vi "Start Logic-Mode dependent case 2.vi"(6 "Case name string":string, 8 "error in (no error)":errorcluster, 9 "cancelled":bool, 10 "UI queue":refnum<queue>, 11 "Acq. queue in":refnum<queue>) -> (0 "error out":errorcluster, 3 "Acq. queue out":refnum<queue>)   [LabVIEW 2017]
uses:
  Queue/Message Queue/Typedefs/Message Cluster.ctl
  Typedefs/Read Write Enum.ctl
  Typedefs/Top level VI states.ctl
  Global Variables/gl_UI Ctrl Refs.vi
  Global Variables/General Globals.vi
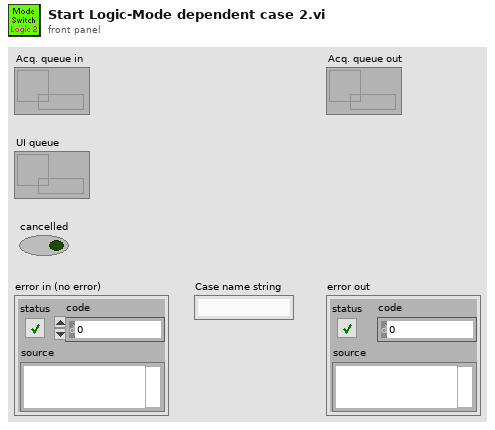
[diagram p1: front panel]
types:
  T1 = typedef "Read Write Enum.ctl" = enum16{"Read", "Write"}
  T2 = typedef "Top level VI states.ctl" = enum16{"None", "Initialise UI", "<STACK PROTOCOL STATES>", "AOL Zstack-START", "AOL Zstack-STOP", "Motor Zstack-START", "Motor Zstack-STOP", "Parameter Sweep-START", "Parameter Sweep-STOP", "<ACQUISITION PROTOCOL STATES> ", "Functional Acquisition-START", "Functional Acquisition-STOP", "Single Plane Acquisition-START", "Single Plane Acquisition-STOP", "Volume Acquisition-START", "Volume Acquisition-STOP", "<LIVE IMAGING PROTOCOL STATES>", "Live Imaging-START", "Live Imaging-STOP", "Live Plane Imaging-START", "Live Plane Imaging-STOP", "Live Volume Imaging-START", "Live Volume Imaging-STOP", "<MOVEMENT CORRECTION PROTOCOL STATES>", "EXIT"}
  T3 = typedef "UI ctrl refs cluster.ctl" = cluster{"Top level VI path":path, "Top level VI ref":refnum<vi>, "User menu ref":refnum<k9>, "Sub Panel control":refnum<vi>, "Imaging Param Tab":refnum<vi>, "Occurrence-Start drivers":refnum<k4>, "Occurrence-Speed logging initialised":refnum<k4>, "Occurrence-XYZ stage initialised":refnum<k4>, "Exit button":refnum<vi>, "Status ind":refnum<vi>, "Set as origin":refnum<vi>, "Speed Logging":refnum<vi>, "Time Lapse":refnum<vi>, "Live Imaging":refnum<vi>, "AOL Z Stack":refnum<vi>, "Motor Z Stack":refnum<vi>, "Funct Acq button":refnum<vi>, "Hard Shutter":refnum<vi>, "Virtual Shutter":refnum<vi>, "Laser Power":refnum<vi>, "AOL Mode":refnum<vi>, "Frame Size":refnum<vi>, "Field of View":refnum<vi>, "Dwell Time":refnum<vi>, "Zoom":refnum<vi>, "AOL Z":refnum<vi>, "Objective":refnum<vi>, "Axis":refnum<vi>, "Paths & Names":refnum<vi>, "Experiment folder path (ind.)":refnum<vi>, "Last State (Ind.)":refnum<vi>, "Averages":refnum<vi>, "Angle (degrees)":refnum<vi>, "X centre":refnum<vi>, "Y centre":refnum<vi>, "Plane Mode":refnum<vi>, "# Planes":refnum<vi>, "Z Start":refnum<vi>, "Z Stop":refnum<vi>, "Z Step":refnum<vi>, "PMT 1":refnum<vi>, "PMT 2":refnum<vi>, "Stage XYZ Position":refnum<vi>, "Pockels@Z Start":refnum<vi>, "Pockels@Z Stop":refnum<vi>, "Obtain Z Start":refnum<vi>, "Obtain Z Stop":refnum<vi>, "Live stim.trig.period":refnum<vi>, "Live stim.trig.enable":refnum<vi>, "Movement Correction":refnum<vi>, "Load Reference Image":refnum<vi>, "XY Stage Move":refnum<vi>, "MovCor Cluster":refnum<vi>, "RefDAQParam":refnum<vi>, "Funct. Acq. Pockels Modulation":refnum<vi>, "Ref Laser Power":refnum<vi>, "Enable Video Recording":refnum<vi>, "Video Record-Live Imaging":refnum<vi>, "Video Record-Funct acq":refnum<vi>, "Reference Source":refnum<vi>, "AOL Z-stack Chirps Ready (ind)":refnum<vi>, "Target time between mov.cor. ref triggers (ms)":refnum<vi>, "Funct. Acq. Ref frame save":refnum<vi>, "Tracking button":refnum<vi>, "Show ref plots window":refnum<vi>, "Center freq ind (nm)":refnum<vi>, "Pickup mode (ind)":refnum<vi>, "Logging queue (ind)":refnum<vi>, "Back aperture power (ind.)":refnum<vi>, "Power after objective (ind.)":refnum<vi>, "Switch user":refnum<vi>, "Ls1 Conn. Status":refnum<vi>, "Ls1Tuning Status":refnum<vi>, "Ls1 Faults":refnum<vi>, "Ls1 Connection":refnum<vi>, "Ls1 Mode":refnum<vi>, "Ls1 POWER [mW]":refnum<vi>, "Ls1Shutter":refnum<vi>, "Ls1 Wavelength":refnum<vi>, "Ls1 Note":refnum<vi>, "Ls1 Confirm Wav":refnum<vi>, "Ls1 PreChrp Prism1":refnum<vi>, "Ls1 PreChrp Prism2":refnum<vi>, "Ls1 wav top Ind":refnum<vi>, "Ls1 power top Ind":refnum<vi>, "Ls1 Pump peak Hold":refnum<vi>, "Ls1 Status Ind":refnum<vi>, "Ls1 wav cancel":refnum<vi>, "Experiment Type":refnum<vi>, "Biology Information":refnum<vi>, "Camera recording status":refnum<vi>, "# Sw. Planes":refnum<vi>, "Sweep Chirps ready":refnum<vi>, "Low-High Resolution Settings":refnum<vi>, "Parameter Sweep":refnum<vi>, "Sweep Chirps ready":refnum<vi>, "Start Sweep":refnum<vi>}
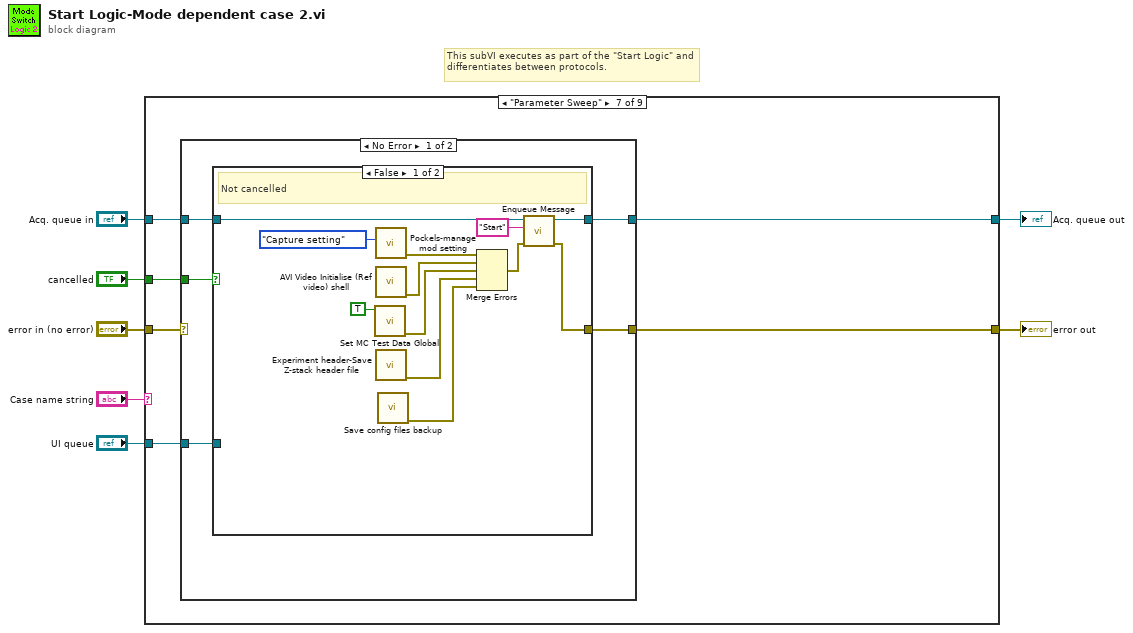
[diagram p0: block diagram]
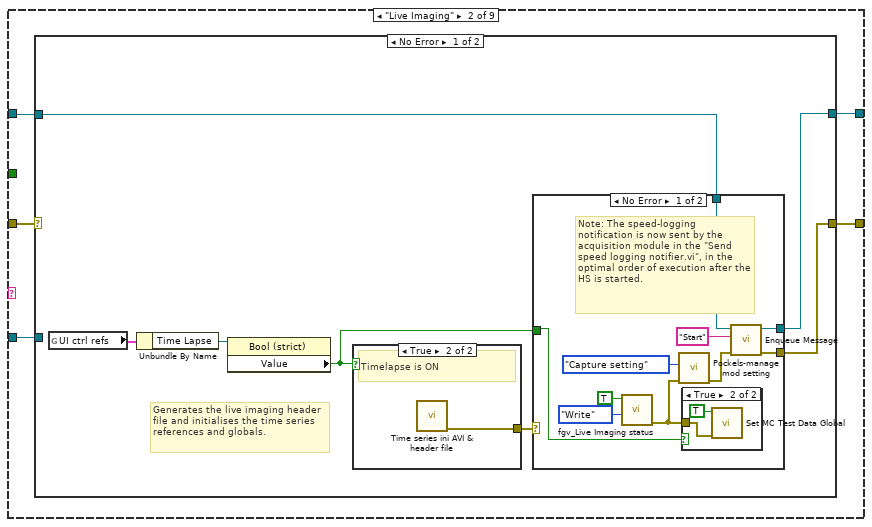
[diagram p3: hidden frame]
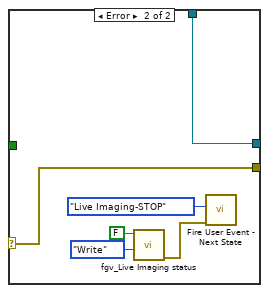
[diagram p5: hidden frame]
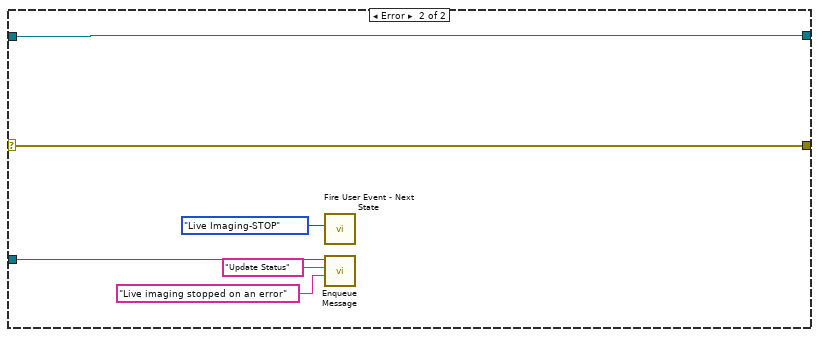
[diagram p7: hidden frame]
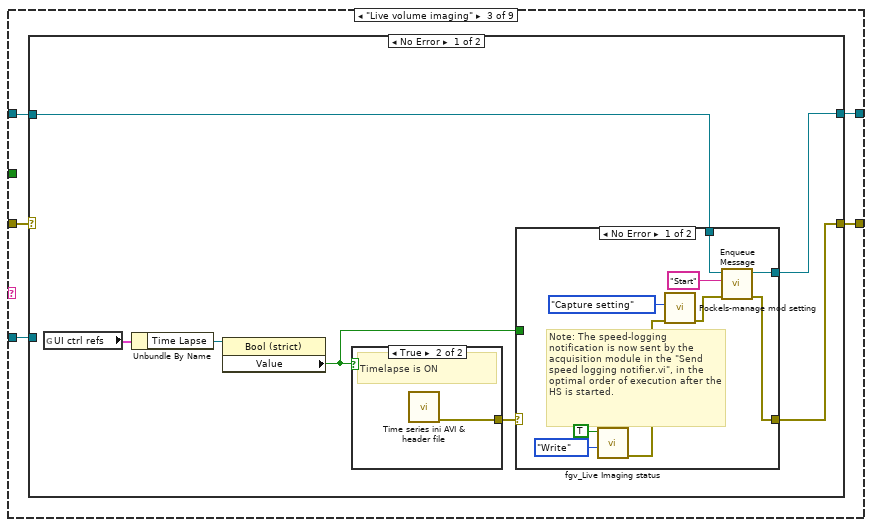
[diagram p8: hidden frame]
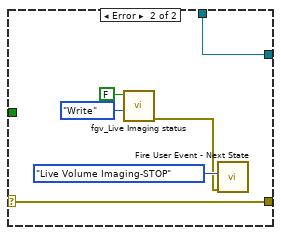
[diagram p9: hidden frame]
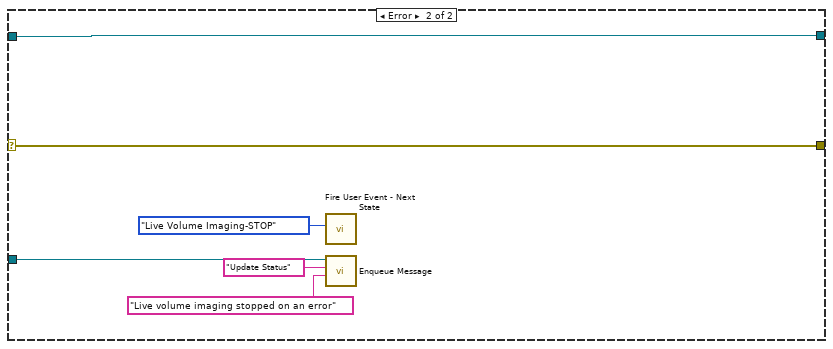
[diagram p11: hidden frame]
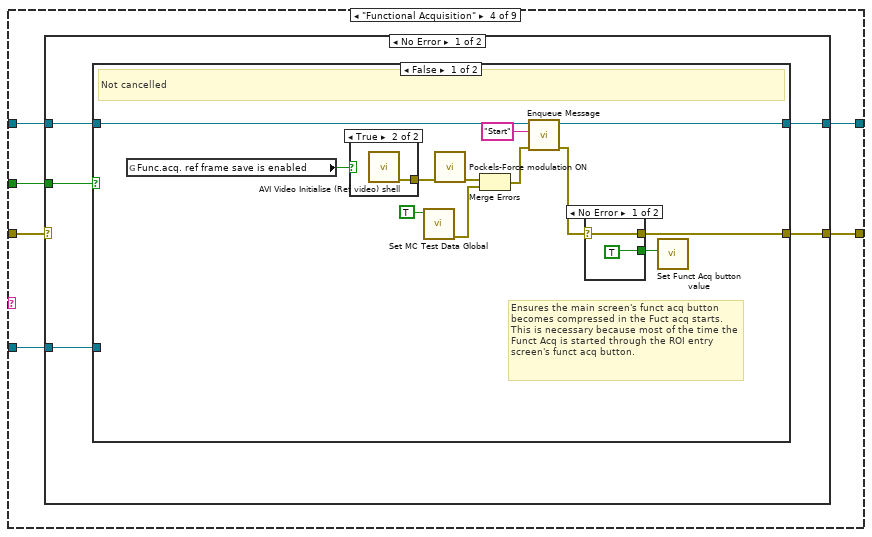
[diagram p12: hidden frame]
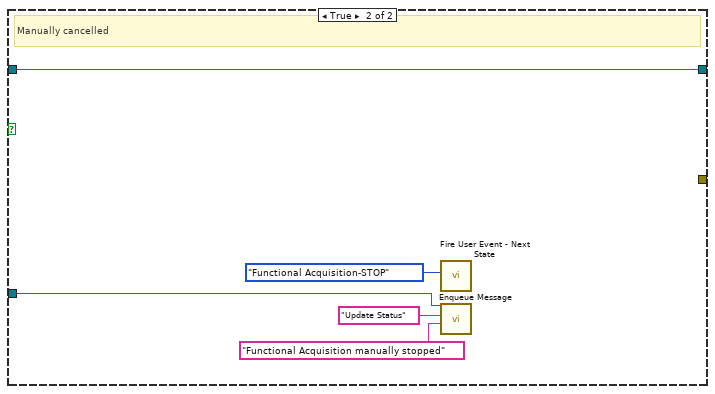
[diagram p15: hidden frame]
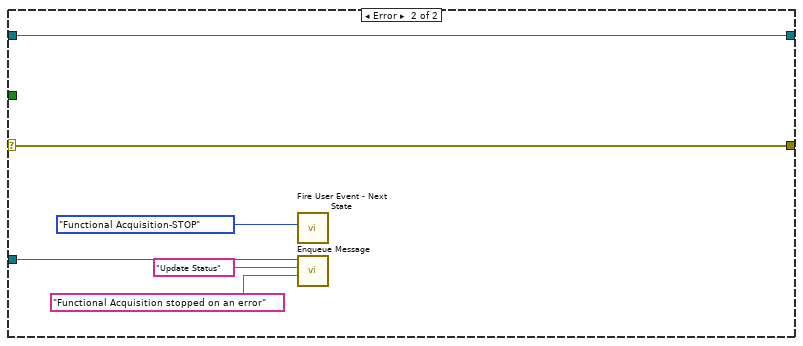
[diagram p16: hidden frame]
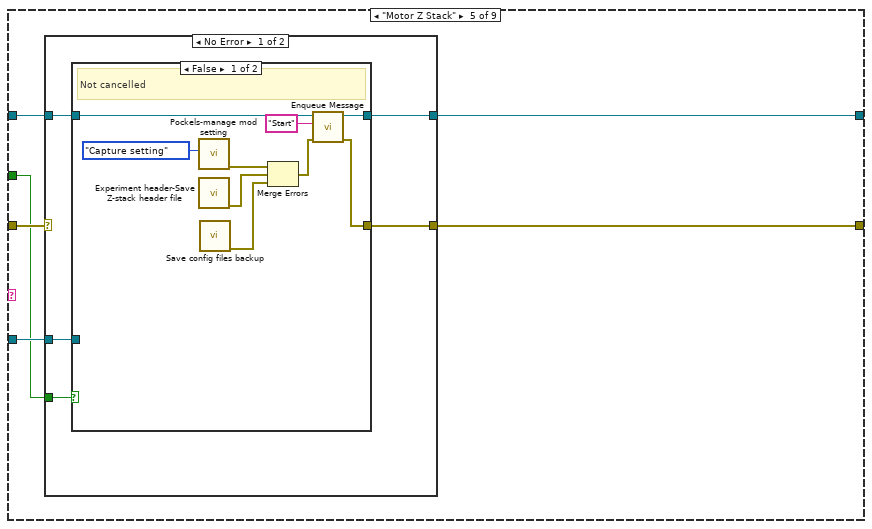
[diagram p17: hidden frame]
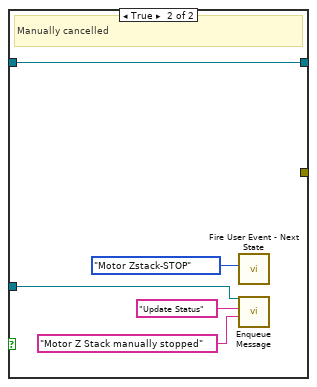
[diagram p18: hidden frame]
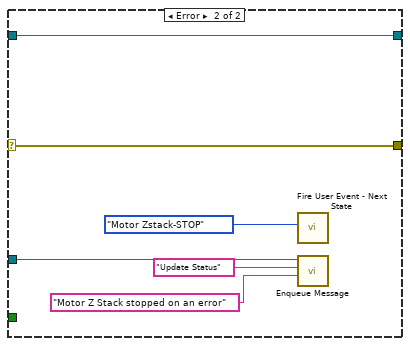
[diagram p19: hidden frame]
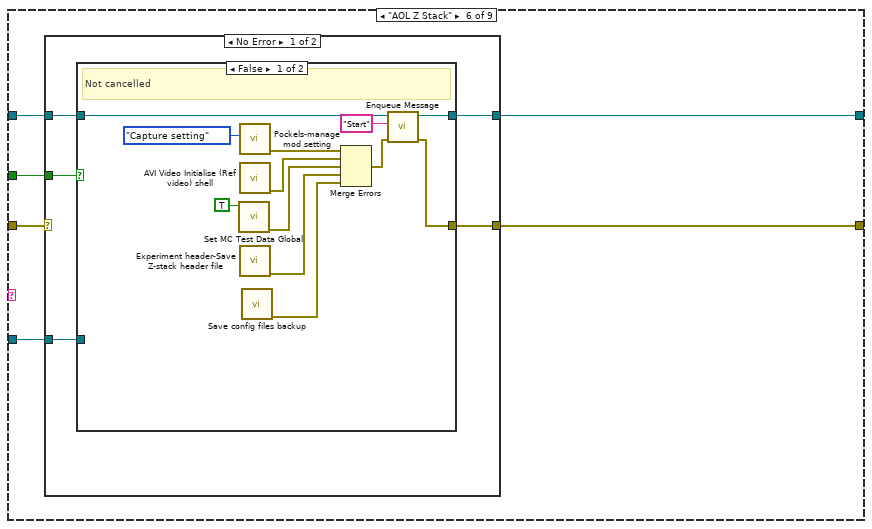
[diagram p20: hidden frame]
diagram:
  # "This subVI executes as part of the \"Start Logic\" and differentiates between protocols."
  n1 = case shown="\"Parameter Sweep\"" "Case name string" {
    tunnel: [w9 w14 w51 w83 w121 w152 w186 w220 w250] -> w1
    tunnel: "error in (no error)" -> [w9 w11 w48 w84 w122 w153 w187 w221 w251]
    tunnel: [w8 w12 w49 w86 w124 w155 w189 w223 w253] -> w3
    tunnel: "Acq. queue in" -> [w8 w13 w50 w85 w123 w154 w188 w222 w252]
    tunnel: "UI queue" -> [_ w10 w47 w82 w120 w151 w185 w219 w249]
    tunnel: "cancelled" -> [_ _ _ w81 w119 w150 w184 w218 w248]
    frame Default {
    }
    frame "Live Imaging" {
      n2 = case shown="No Error" w11 {
        selector: w11 -> [_ w46]
        tunnel: [w16 w46] -> w14
        tunnel: w13 -> [w18 w45]
        tunnel: [w17 w45] -> w12
        tunnel: w10 -> [_ w41]
        frame No Error {
          # "Generates the live imaging header file and initialises the time series references and globals."
          n3 = global read "gl_UI Ctrl Refs.vi" "UI ctrl refs"() -> (w15:T3)
          n4 = Unbundle By Name(w15) -> ("Time Lapse"=w21:refnum<vi>)
          n5 = property class="Bool (strict)"(reference=w21) -> ("Value"=w19:bool)  [unwired: 1 in, 2 out]
          n6 = case shown="True" w19 {
            tunnel: [_ w40] -> w20
            frame False {
              # "Timelapse is OFF"
            }
            frame True {
              # "Timelapse is ON"
              n7 = call "Time series ini AVI & header file.vi"() -> ("error out"=w40:errorcluster)  [unwired: 11 in]
            }
          }
          n8 = case shown="No Error" w20 {
            selector: w20 -> [_ w37]
            tunnel: w19 -> [w22 _]
            tunnel: w18 -> [w28 w38]
            tunnel: [w30 w38] -> w17
            tunnel: [w29 w37] -> w16
            frame No Error {
              # "Note: The speed-logging notification is now sent by the acquisition module in the \"Send speed logging notifier.vi\", in the optimal order of execution after the HS is started."
              n9 = call "fgv_Live Imaging status.vi"("Function"=Read_Write_Enum."Write", "Live Imaging?"=TRUE ("Timelapse?")) -> ("error out"=w23:errorcluster)  [unwired: 8 in, 1 out]
              n10 = call "Pockels-manage mod setting.vi"("error in (no error)"=w23, "Function"=enum16{"Capture setting", "Re-apply setting"}."Capture setting") -> ("error out"=w27:errorcluster)  [unwired: 9 in]
              n11 = case shown="True" w22 {
                tunnel: w23 -> [_ w32]
                frame False {
                }
                frame True {
                  n12 = call "Set MC Test Data Global.vi"("error in (no error)"=w32, "Save MC TestData"=TRUE) -> ()  [unwired: 8 in, 2 out]
                }
              }
              n13 = call "Enqueue Message.vi"("error in (no error)"=w27, "Message"="Start", "Queue"=w28) -> ("error out"=w29:errorcluster, "Queue out"=w30:refnum<queue>)  [unwired: 7 in]
            }
            frame Error {
              n14 = call "fgv_Live Imaging status.vi"("Function"=Read_Write_Enum."Write", "Live Imaging?"=FALSE ("Timelapse?")) -> ("error out"=w34:errorcluster)  [unwired: 8 in, 1 out]
              n15 = call "Fire User Event - Next State.vi"("Error In"=w34, "\"UI Handler loop\" case to execute"=Top_level_VI_states."Live Imaging-STOP" ("event data / imaging mode")) -> ()  [unwired: 9 in, 1 out]
            }
          }
        }
        frame Error {
          n16 = call "Fire User Event - Next State.vi"("\"UI Handler loop\" case to execute"=Top_level_VI_states."Live Imaging-STOP" ("event data / imaging mode")) -> ()  [unwired: 10 in, 1 out]
          n17 = call "Enqueue Message.vi"("Message Data"="Live imaging stopped on an error" ("Acquiring and Logging..."), "Message"="Update Status", "Queue"=w41) -> ()  [unwired: 7 in, 2 out]
        }
      }
    }
    frame "Live volume imaging" {
      n18 = case shown="No Error" w48 {
        selector: w48 -> [_ w80]
        tunnel: [w55 w80] -> w51
        tunnel: w50 -> [w54 w79]
        tunnel: [w53 w79] -> w49
        tunnel: w47 -> [_ w76]
        frame No Error {
          n19 = global read "gl_UI Ctrl Refs.vi" "UI ctrl refs"() -> (w52:T3)
          n20 = Unbundle By Name(w52) -> ("Time Lapse"=w58:refnum<vi>)
          n21 = property class="Bool (strict)"(reference=w58) -> ("Value"=w56:bool)  [unwired: 1 in, 2 out]
          n22 = case shown="True" w56 {
            tunnel: [_ w74] -> w57
            frame False {
              # "Timelapse is OFF"
            }
            frame True {
              # "Timelapse is ON"
              n23 = call "Time series ini AVI & header file.vi"() -> ("error out"=w74:errorcluster)  [unwired: 11 in]
            }
          }
          n24 = case shown="No Error" w57 {
            selector: w57 -> [_ w73]
            tunnel: [w66 w73] -> w55
            tunnel: w56 -> [_ _]
            tunnel: w54 -> [w65 w71]
            tunnel: [w64 w71] -> w53
            frame No Error {
              # "Note: The speed-logging notification is now sent by the acquisition module in the \"Send speed logging notifier.vi\", in the optimal order of execution after the HS is started."
              n25 = call "fgv_Live Imaging status.vi"("Function"=Read_Write_Enum."Write", "Live Imaging?"=TRUE ("Timelapse?")) -> ("error out"=w59:errorcluster)  [unwired: 8 in, 1 out]
              n26 = call "Pockels-manage mod setting.vi"("error in (no error)"=w59, "Function"=enum16{"Capture setting", "Re-apply setting"}."Capture setting") -> ("error out"=w63:errorcluster)  [unwired: 9 in]
              n27 = call "Enqueue Message.vi"("error in (no error)"=w63, "Message"="Start", "Queue"=w65) -> ("error out"=w66:errorcluster, "Queue out"=w64:refnum<queue>)  [unwired: 7 in]
            }
            frame Error {
              n28 = call "fgv_Live Imaging status.vi"("Function"=Read_Write_Enum."Write", "Live Imaging?"=FALSE ("Timelapse?")) -> ("error out"=w68:errorcluster)  [unwired: 8 in, 1 out]
              n29 = call "Fire User Event - Next State.vi"("Error In"=w68, "\"UI Handler loop\" case to execute"=Top_level_VI_states."Live Volume Imaging-STOP" ("event data / imaging mode")) -> ()  [unwired: 9 in, 1 out]
            }
          }
        }
        frame Error {
          n30 = call "Fire User Event - Next State.vi"("\"UI Handler loop\" case to execute"=Top_level_VI_states."Live Volume Imaging-STOP" ("event data / imaging mode")) -> ()  [unwired: 10 in, 1 out]
          n31 = call "Enqueue Message.vi"("Message Data"="Live volume imaging stopped on an error" ("Acquiring and Logging..."), "Message"="Update Status", "Queue"=w76) -> ()  [unwired: 7 in, 2 out]
        }
      }
    }
    frame "Functional Acquisition" {
      n32 = case shown="No Error" w84 {
        selector: w84 -> [_ w117]
        tunnel: [w87 w117] -> w83
        tunnel: [w88 w118] -> w86
        tunnel: w85 -> [w89 w118]
        tunnel: w82 -> [w91 w113]
        tunnel: w81 -> [w90 _]
        frame No Error {
          n33 = case shown="False" w90 {
            tunnel: w91 -> [_ w109]
            tunnel: w89 -> [w102 w108]
            tunnel: [w101 w108] -> w88
            tunnel: [w93 _] -> w87
            frame False {
              # "Ensures the main screen's funct acq button becomes compressed in the Fuct acq starts. This is necessary because most of the time the Funct Acq is started through the ROI entry screen's funct acq button."
              # "Not cancelled"
              n34 = global read "General Globals.vi" "Func.acq. ref frame save is enabled"() -> (w95:bool)
              n35 = case shown="True" w95 {
                tunnel: [_ w107] -> w100
                frame False {
                }
                frame True {
                  n36 = call "AVI Video Initialise (Ref video) shell.vi"() -> ("error out"=w107:errorcluster)  [unwired: 11 in]
                }
              }
              n37 = call "Set MC Test Data Global.vi"("Save MC TestData"=TRUE) -> ("error out"=w98:errorcluster)  [unwired: 9 in, 1 out]
              n38 = call "Pockels-Force modulation ON.vi"("error in (no error)"=w100) -> ("error out"=w97:errorcluster)  [unwired: 10 in]
              n39 = Merge Errors(w97, w98) -> (w96:errorcluster)
              n40 = call "Enqueue Message.vi"("error in (no error)"=w96, "Message"="Start", "Queue"=w102) -> ("error out"=w94:errorcluster, "Queue out"=w101:refnum<queue>)  [unwired: 7 in]
              n41 = case shown="No Error" w94 {
                selector: w94 -> [w105 w106]
                tunnel: [w105 w106] -> w93
                tunnel: [TRUE ("Value") _] -> w92
                frame No Error {
                }
                frame Error {
                }
              }
              n42 = call "Set Funct Acq button value.vi"("Functional Acquisition button's new value"=w92) -> ()  [unwired: 10 in, 1 out]
            }
            frame True {
              # "Manually cancelled"
              n43 = call "Fire User Event - Next State.vi"("\"UI Handler loop\" case to execute"=Top_level_VI_states."Functional Acquisition-STOP" ("event data / imaging mode")) -> ()  [unwired: 10 in, 1 out]
              n44 = call "Enqueue Message.vi"("Message Data"="Functional Acquisition manually stopped" ("Acquiring and Logging..."), "Message"="Update Status", "Queue"=w109) -> ()  [unwired: 7 in, 2 out]
            }
          }
        }
        frame Error {
          n45 = call "Fire User Event - Next State.vi"("\"UI Handler loop\" case to execute"=Top_level_VI_states."Functional Acquisition-STOP" ("event data / imaging mode")) -> ()  [unwired: 10 in, 1 out]
          n46 = call "Enqueue Message.vi"("Message Data"="Functional Acquisition stopped on an error" ("Acquiring and Logging..."), "Message"="Update Status", "Queue"=w113) -> ()  [unwired: 7 in, 2 out]
        }
      }
    }
    frame "Motor Z Stack" {
      n47 = case shown="No Error" w122 {
        selector: w122 -> [_ w148]
        tunnel: [w125 w148] -> w121
        tunnel: [w126 w149] -> w124
        tunnel: w123 -> [w127 w149]
        tunnel: w120 -> [w129 w144]
        tunnel: w119 -> [w128 _]
        frame No Error {
          n48 = case shown="False" w128 {
            tunnel: w129 -> [_ w140]
            tunnel: w127 -> [w137 w139]
            tunnel: [w136 w139] -> w126
            tunnel: [w135 _] -> w125
            frame False {
              # "Not cancelled"
              n49 = call "Pockels-manage mod setting.vi"("Function"=enum16{"Capture setting", "Re-apply setting"}."Capture setting") -> ("error out"=w133:errorcluster)  [unwired: 10 in]
              n50 = call "Experiment header-Save Z-stack header file.vi"() -> ("error out"=w132:errorcluster)  [unwired: 10 in, 1 out]
              n51 = call "Save config files backup.vi"() -> ("error out"=w130:errorcluster)  [unwired: 11 in]
              n52 = Merge Errors(w133, w132, w130) -> (w131:errorcluster)
              n53 = call "Enqueue Message.vi"("error in (no error)"=w131, "Message"="Start", "Queue"=w137) -> ("error out"=w135:errorcluster, "Queue out"=w136:refnum<queue>)  [unwired: 7 in]
            }
            frame True {
              # "Manually cancelled"
              n54 = call "Fire User Event - Next State.vi"("\"UI Handler loop\" case to execute"=Top_level_VI_states."Motor Zstack-STOP" ("event data / imaging mode")) -> ()  [unwired: 10 in, 1 out]
              n55 = call "Enqueue Message.vi"("Message Data"="Motor Z Stack manually stopped" ("Acquiring and Logging..."), "Message"="Update Status", "Queue"=w140) -> ()  [unwired: 7 in, 2 out]
            }
          }
        }
        frame Error {
          n56 = call "Fire User Event - Next State.vi"("\"UI Handler loop\" case to execute"=Top_level_VI_states."Motor Zstack-STOP" ("event data / imaging mode")) -> ()  [unwired: 10 in, 1 out]
          n57 = call "Enqueue Message.vi"("Message Data"="Motor Z Stack stopped on an error" ("Acquiring and Logging..."), "Message"="Update Status", "Queue"=w144) -> ()  [unwired: 7 in, 2 out]
        }
      }
    }
    frame "AOL Z Stack" {
      n58 = case shown="No Error" w153 {
        selector: w153 -> [_ w182]
        tunnel: [w156 w182] -> w152
        tunnel: [w157 w183] -> w155
        tunnel: w154 -> [w158 w183]
        tunnel: w151 -> [w160 w178]
        tunnel: w150 -> [w159 _]
        frame No Error {
          n59 = case shown="False" w159 {
            tunnel: w160 -> [_ w174]
            tunnel: w158 -> [w171 w173]
            tunnel: [w170 w173] -> w157
            tunnel: [w169 _] -> w156
            frame False {
              # "Not cancelled"
              n60 = call "Set MC Test Data Global.vi"("Save MC TestData"=TRUE) -> ("error out"=w163:errorcluster)  [unwired: 9 in, 1 out]
              n61 = call "Pockels-manage mod setting.vi"("Function"=enum16{"Capture setting", "Re-apply setting"}."Capture setting") -> ("error out"=w167:errorcluster)  [unwired: 10 in]
              n62 = call "AVI Video Initialise (Ref video) shell.vi"() -> ("error out"=w165:errorcluster)  [unwired: 11 in]
              n63 = call "Experiment header-Save Z-stack header file.vi"() -> ("error out"=w162:errorcluster)  [unwired: 10 in, 1 out]
              n64 = call "Save config files backup.vi"() -> ("error out"=w161:errorcluster)  [unwired: 11 in]
              n65 = Merge Errors(w167, w165, w163, w162, w161) -> (w166:errorcluster)
              n66 = call "Enqueue Message.vi"("error in (no error)"=w166, "Message"="Start", "Queue"=w171) -> ("error out"=w169:errorcluster, "Queue out"=w170:refnum<queue>)  [unwired: 7 in]
            }
            frame True {
              # "Manually cancelled"
              n67 = call "Fire User Event - Next State.vi"("\"UI Handler loop\" case to execute"=Top_level_VI_states."AOL Zstack-STOP" ("event data / imaging mode")) -> ()  [unwired: 10 in, 1 out]
              n68 = call "Enqueue Message.vi"("Message Data"="AOL Z Stack manually stopped" ("Acquiring and Logging..."), "Message"="Update Status", "Queue"=w174) -> ()  [unwired: 7 in, 2 out]
            }
          }
        }
        frame Error {
          n69 = call "Fire User Event - Next State.vi"("\"UI Handler loop\" case to execute"=Top_level_VI_states."AOL Zstack-STOP" ("event data / imaging mode")) -> ()  [unwired: 10 in, 1 out]
          n70 = call "Enqueue Message.vi"("Message Data"="AOL Z Stack stopped on an error" ("Acquiring and Logging..."), "Message"="Update Status", "Queue"=w178) -> ()  [unwired: 7 in, 2 out]
        }
      }
    }
    frame "Parameter Sweep" {
      n71 = case shown="No Error" w187 {
        selector: w187 -> [_ w216]
        tunnel: [w190 w216] -> w186
        tunnel: [w191 w217] -> w189
        tunnel: w188 -> [w192 w217]
        tunnel: w185 -> [w194 w212]
        tunnel: w184 -> [w193 _]
        frame No Error {
          n72 = case shown="False" w193 {
            tunnel: w194 -> [_ w208]
            tunnel: w192 -> [w205 w207]
            tunnel: [w204 w207] -> w191
            tunnel: [w203 _] -> w190
            frame False {
              # "Not cancelled"
              n73 = call "Set MC Test Data Global.vi"("Save MC TestData"=TRUE) -> ("error out"=w197:errorcluster)  [unwired: 9 in, 1 out]
              n74 = call "Pockels-manage mod setting.vi"("Function"=enum16{"Capture setting", "Re-apply setting"}."Capture setting") -> ("error out"=w201:errorcluster)  [unwired: 10 in]
              n75 = call "AVI Video Initialise (Ref video) shell.vi"() -> ("error out"=w199:errorcluster)  [unwired: 11 in]
              n76 = call "Experiment header-Save Z-stack header file.vi"() -> ("error out"=w196:errorcluster)  [unwired: 10 in, 1 out]
              n77 = call "Save config files backup.vi"() -> ("error out"=w195:errorcluster)  [unwired: 11 in]
              n78 = Merge Errors(w201, w199, w197, w196, w195) -> (w200:errorcluster)
              n79 = call "Enqueue Message.vi"("error in (no error)"=w200, "Message"="Start", "Queue"=w205) -> ("error out"=w203:errorcluster, "Queue out"=w204:refnum<queue>)  [unwired: 7 in]
            }
            frame True {
              # "Manually cancelled"
              n80 = call "Fire User Event - Next State.vi"("\"UI Handler loop\" case to execute"=Top_level_VI_states."Parameter Sweep-STOP" ("event data / imaging mode")) -> ()  [unwired: 10 in, 1 out]
              n81 = call "Enqueue Message.vi"("Message Data"="Parameter Sweep manually stopped" ("Acquiring and Logging..."), "Message"="Update Status", "Queue"=w208) -> ()  [unwired: 7 in, 2 out]
            }
          }
        }
        frame Error {
          n82 = call "Fire User Event - Next State.vi"("\"UI Handler loop\" case to execute"=Top_level_VI_states."Parameter Sweep-STOP" ("event data / imaging mode")) -> ()  [unwired: 10 in, 1 out]
          n83 = call "Enqueue Message.vi"("Message Data"="Parameter sweep stopped on an error" ("Acquiring and Logging..."), "Message"="Update Status", "Queue"=w212) -> ()  [unwired: 7 in, 2 out]
        }
      }
    }
    frame "Volume acquisition" {
      n84 = case shown="No Error" w221 {
        selector: w221 -> [_ w246]
        tunnel: [w224 w246] -> w220
        tunnel: [w225 w247] -> w223
        tunnel: w222 -> [w226 w247]
        tunnel: w219 -> [w228 w242]
        tunnel: w218 -> [w227 _]
        frame No Error {
          n85 = case shown="False" w227 {
            tunnel: w228 -> [_ w238]
            tunnel: w226 -> [w235 w237]
            tunnel: [w234 w237] -> w225
            tunnel: [w233 _] -> w224
            frame False {
              # "Not cancelled"
              n86 = call "AVI Video Initialise (Ref video) shell.vi"() -> ("error out"=w230:errorcluster)  [unwired: 11 in]
              n87 = call "Set MC Test Data Global.vi"("Save MC TestData"=TRUE) -> ("error out"=w231:errorcluster)  [unwired: 9 in, 1 out]
              n88 = Merge Errors(w230, w231) -> (w229:errorcluster)
              n89 = call "Enqueue Message.vi"("error in (no error)"=w229, "Message"="Start", "Queue"=w235) -> ("error out"=w233:errorcluster, "Queue out"=w234:refnum<queue>)  [unwired: 7 in]
            }
            frame True {
              # "Manually cancelled"
              n90 = call "Fire User Event - Next State.vi"("\"UI Handler loop\" case to execute"=Top_level_VI_states."Volume Acquisition-STOP" ("event data / imaging mode")) -> ()  [unwired: 10 in, 1 out]
              n91 = call "Enqueue Message.vi"("Message Data"="Volume Acquisition manually stopped" ("Acquiring and Logging..."), "Message"="Update Status", "Queue"=w238) -> ()  [unwired: 7 in, 2 out]
            }
          }
        }
        frame Error {
          n92 = call "Fire User Event - Next State.vi"("\"UI Handler loop\" case to execute"=Top_level_VI_states."Volume Acquisition-STOP" ("event data / imaging mode")) -> ()  [unwired: 10 in, 1 out]
          n93 = call "Enqueue Message.vi"("Message Data"="Volume Acquisition stopped on an error" ("Acquiring and Logging..."), "Message"="Update Status", "Queue"=w242) -> ()  [unwired: 7 in, 2 out]
        }
      }
    }
    frame "Single Plane Acquisition" {
      n94 = case shown="No Error" w251 {
        selector: w251 -> [_ w276]
        tunnel: [w254 w276] -> w250
        tunnel: [w255 w277] -> w253
        tunnel: w252 -> [w256 w277]
        tunnel: w249 -> [w258 w272]
        tunnel: w248 -> [w257 _]
        frame No Error {
          n95 = case shown="True" w257 {
            tunnel: w258 -> [_ w268]
            tunnel: w256 -> [w265 w267]
            tunnel: [w264 w267] -> w255
            tunnel: [w263 _] -> w254
            frame False {
              # "Not cancelled"
              n96 = call "Pockels-manage mod setting.vi"("Function"=enum16{"Capture setting", "Re-apply setting"}."Capture setting") -> ("error out"=w261:errorcluster)  [unwired: 10 in]
              n97 = call "AVI Video Initialise (Ref video) shell.vi"() -> ("error out"=w260:errorcluster)  [unwired: 11 in]
              n98 = Merge Errors(w261, w260) -> (w259:errorcluster)
              n99 = call "Enqueue Message.vi"("error in (no error)"=w259, "Message"="Start", "Queue"=w265) -> ("error out"=w263:errorcluster, "Queue out"=w264:refnum<queue>)  [unwired: 7 in]
            }
            frame True {
              # "Manually cancelled"
              n100 = call "Fire User Event - Next State.vi"("\"UI Handler loop\" case to execute"=Top_level_VI_states."Single Plane Acquisition-STOP" ("event data / imaging mode")) -> ()  [unwired: 10 in, 1 out]
              n101 = call "Enqueue Message.vi"("Message Data"="Single Plane Acquisition manually stopped" ("Acquiring and Logging..."), "Message"="Update Status", "Queue"=w268) -> ()  [unwired: 7 in, 2 out]
            }
          }
        }
        frame Error {
          n102 = call "Fire User Event - Next State.vi"("\"UI Handler loop\" case to execute"=Top_level_VI_states."Single Plane Acquisition-STOP" ("event data / imaging mode")) -> ()  [unwired: 10 in, 1 out]
          n103 = call "Enqueue Message.vi"("Message Data"="Single Plane Acquisition stopped on an error" ("Acquiring and Logging..."), "Message"="Update Status", "Queue"=w272) -> ()  [unwired: 7 in, 2 out]
        }
      }
    }
  }
  "Acq. queue out" <- w3
  "error out" <- w1
